vi "Dynamic Launch CaseSelect.vi"(8 "error in (no error)":errorcluster, 10 "Owning VI Details":T1) -> (0 "error out":errorcluster)   [LabVIEW 2020]
uses:
  JKI State Machine API/source/JKI SM/JKI SM.lvclass
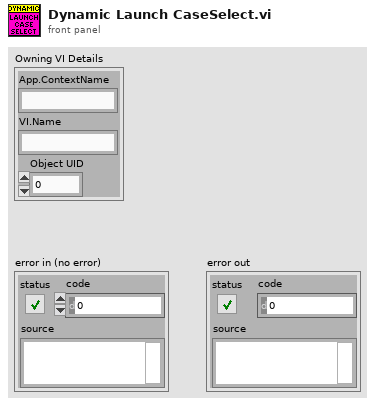
[diagram p1: front panel]
types:
  T1 = cluster{"App.ContextName":string, "VI.Name":string, "Object UID":i32}
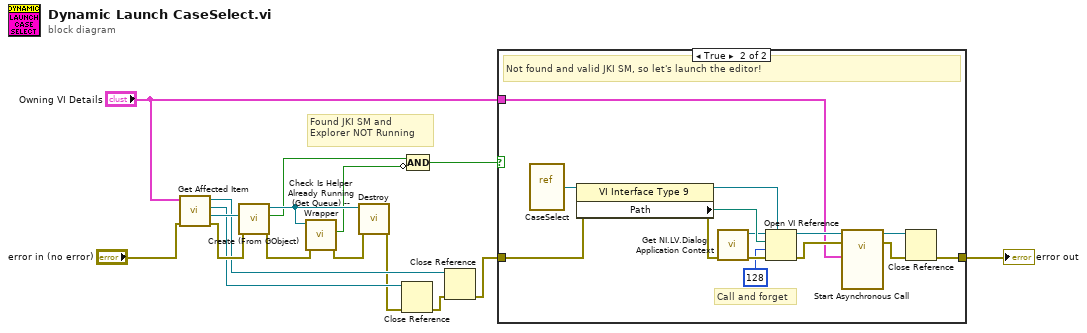
[diagram p0: block diagram]
diagram:
  # "Found JKI SM and Explorer NOT Running"
  n1 = call "Get Affected Item.vi"("error in (no error)"="error in (no error)", "Owning VI Details"="Owning VI Details") -> ("error out"=w6:errorcluster, "GObject"=w8:refnum<vi>, "Owning VI"=w5:refnum<vi>, "Application"=w4:refnum<vi>)  [unwired: 6 in]
  n2 = call "Create (From GObject).vi"("error in (no error)"=w6, "GObject"=w8) -> ("error out"=w15:errorcluster, "Found JKI SMs?"=w12:bool, "JKI SM out"=w13:refnum<class "JKI SM.lvclass">)  [unwired: 6 in, 1 out]
  n3 = call "Check Is Helper Already Running (Get Queue) -- Wrapper.vi"("error in (no error)"=w15, "JKI SM in"=w13) -> ("error out"=w14:errorcluster, "is Running?"=w11:bool)  [unwired: 8 in]
  n4 = call "Destroy.vi"("error in (no error)"=w14, "JKI SM in"=w13) -> ("error out"=w2:errorcluster)  [unwired: 9 in]
  n5 = Close Reference(reference=w5, error in (no error)=w2) -> (error out=w3:errorcluster)
  n6 = Compound Arithmetic op=AND(w12, invert w11) -> (w10:bool)
  n7 = Close Reference(reference=w4, error in (no error)=w3) -> (error out=w1:errorcluster)
  n8 = case shown="True" w10 {
    tunnel: w1 -> [w17 w25]
    tunnel: "Owning VI Details" -> [_ w18]
    tunnel: [w17 w20] -> w16
    frame False {
      # "Don't launch another copy"
    }
    frame True {
      # "Call and forget"
      # "Not found and valid JKI SM, so let's launch the editor!"
      n9 = vi-ref "CaseSelect.vi"() -> (w31:refnum<vi>)
      n10 = property class="VI Interface Type 9"(reference=w31, error in=w25) -> (reference out=w29:refnum<vi>, error out=w24:errorcluster, "Path"=w30:path)
      n11 = call "Get NI.LV.Dialog Application Context.vi"("error in (no error)"=w24) -> ("error out"=w23:errorcluster, "Application out"=w22:refnum<vi>)  [unwired: 9 in]
      n12 = Open VI Reference(type specifier VI Refnum (for type only)=w29, application reference (local)=w22, vi path=w30, options=128, error in (no error)=w23) -> (vi reference=w28:refnum<vi>, error out=w19:errorcluster)  [unwired: 1 in]
      n13 = call-by-ref "Start Asynchronous Call"(reference=w28, error in=w19, "Owning VI Details"=w18) -> (reference out=w27:refnum<vi>, error out=w26:errorcluster)  [unwired: 11 in]
      n14 = Close Reference(reference=w27, error in (no error)=w26) -> (error out=w20:errorcluster)
    }
  }
  "error out" <- w16
